vi "ODBC-32-windows.vi"(8 "error in (no error)":errorcluster caption="错误输入（无错误）", 11 "Database_access 输入":refnum<class "Database_access.lvclass">) -> (0 "error out":errorcluster caption="错误输出", 3 "Database_access 输出":refnum<class "Database_access.lvclass">)   [LabVIEW 2025, in "Database_access.lvclass"]
uses:
  Database_access.lvclass
  Database_access.lvclass/Database_access.ctl
  <vilib>/addons/database/Connection.llb/DB Tools Open Connec (String).vi
  <vilib>/addons/database/NI_Database_API.lvlib
panel:
  # "ODBC 数据源管理系统"
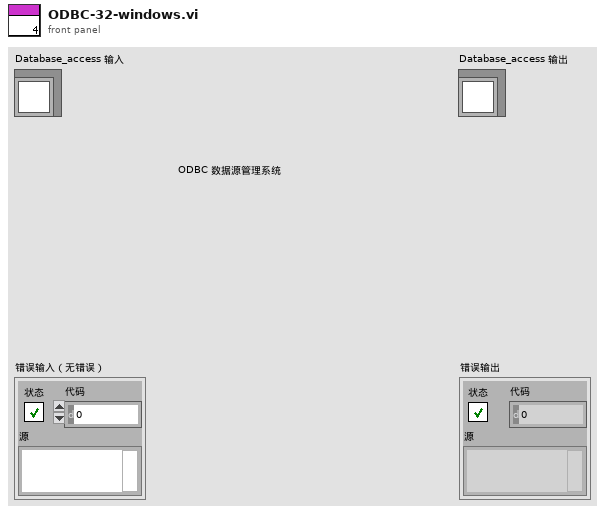
[diagram p1: front panel]
types:
  T1 = typedef "NI_Database_API.lvlib/Conn ObjectReference.ctl" = refnum<k1>
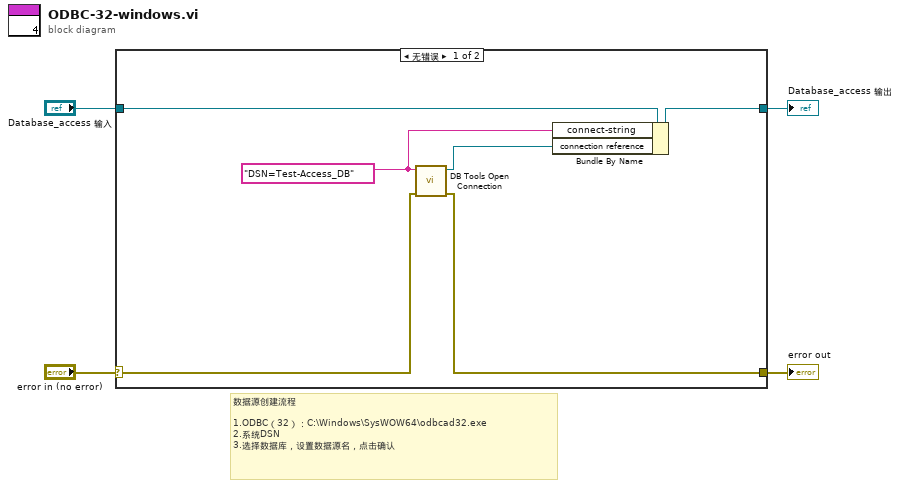
[diagram p0: block diagram]
diagram:
  # "数据源创建流程\n\n1.ODBC（32）：C:\\Windows\\SysWOW64\\odbcad32.exe\n2.系统DSN\n3.选择数据库，设置数据源名，点击确认"
  n1 = case shown="无错误" "error in (no error)" {
    selector: "error in (no error)" -> [w5 w12]
    tunnel: [w6 w12] -> w3
    tunnel: [w9 w11] -> w1
    tunnel: "Database_access 输入" -> [w10 w11]
    frame No Error {
      w8 = "DSN=Test-Access_DB"
      n2 = call-poly <vilib>:"DB Tools Open Connection.vi"("error in (no error)"=w5, "connection information"=w8) -> ("error out"=w6:errorcluster, "connection reference"=w7:T1)  [unwired: 6 in]
      n3 = Bundle By Name(cluster=w10, "connect-string"=w8, "connection reference"=w7) -> (w9:refnum<class "Database_access.lvclass">)
    }
    frame Error {
    }
  }
  "error out" <- w3
  "Database_access 输出" <- w1
